vi "Context Owner.vi"() -> ()   [LabVIEW 2019, in "RemoteControl.ZMQ.lvlib" / "ZMQ.ContextManager.lvlib"]
uses:
  ZMQ.ContextManager.lvlib
  Typedefs/Action--enum.ctl
  <vilib>/addons/zeromq/zmq_context.lvclass
panel:
  out "Numeric":i32
  in  "stop":bool
  out "error out":errorcluster
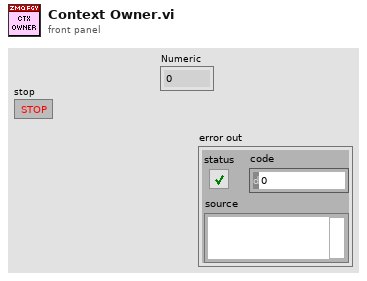
[diagram p1: front panel]
types:
  T1 = typedef "RemoteControl.ZMQ.lvlib/ZMQ.ContextManager.lvlib/Action--enum.ctl" = enum16{"Get Context", "Release Context", "Socket Opened", "Socket Closed", "Force Cleanup", "Set Context", "Retire If Idle"}
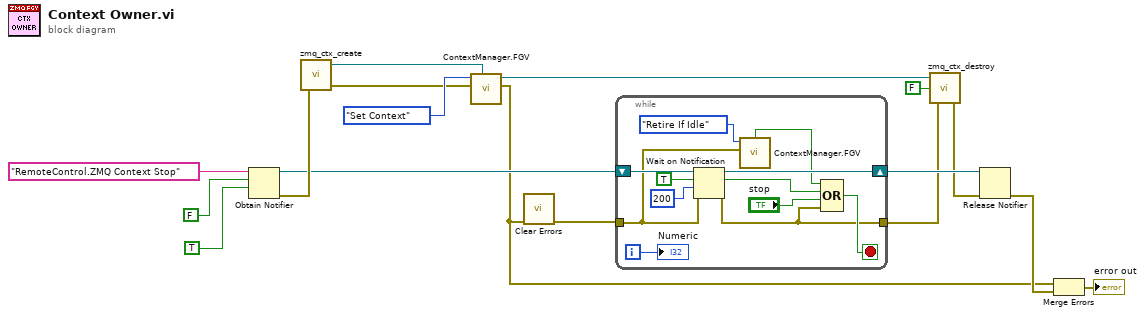
[diagram p0: block diagram]
diagram:
  n1 = Obtain Notifier(name (unnamed)="RemoteControl.ZMQ Context Stop", notification data type=FALSE, create if not found? (T)=TRUE) -> (notifier out=w5:refnum<notifier>, error out=w6:errorcluster)  [unwired: 1 in, 1 out]
  n2 = call <vilib>:"zmq_ctx_create.vi"("error in"=w6) -> ("error out"=w12:errorcluster, "context out"=w14:refnum<class "zmq_context.lvclass">)  [unwired: 3 in]
  n3 = call "ContextManager.FGV.vi"("context in"=w14, "error in"=w12, "action"=Action--enum."Set Context") -> ("error out"=w2:errorcluster, "context out"=w1:refnum<class "zmq_context.lvclass">)  [unwired: 6 in, 1 out]
  n4 = call <vilib>:"Clear Errors.vi"("error in (no error)"=w2) -> ("error out"=w7:errorcluster)  [unwired: 5 in, 1 out]
  n5 = while {
    shift-right: [w28] -> w10
    shift-left: w5 -> [w26]
    tunnel: w7 -> [w20]
    tunnel: [w19] -> w4
    i -> [w21]
    stop <- w24 stop-if-true
    n6 = Wait on Notification(notifier=w26, ignore previous (F)=TRUE, timeout in ms (-1)=200, error in (no error)=w20) -> (notifier out=w28:refnum<notifier>, notification=w25:bool, error out=w19:errorcluster)  [unwired: 1 out]
    n7 = call "ContextManager.FGV.vi"("error in"=w20, "action"=Action--enum."Retire If Idle") -> ("retired?"=w23:bool)  [unwired: 7 in, 2 out]
    n8 = Compound Arithmetic op=OR(w23, w25, "stop", w19) -> (w24:bool)
    "Numeric" <- w21
  }
  n9 = call <vilib>:"zmq_ctx_destroy.vi"("error in"=w4, "reap? (F)"=FALSE, "context in"=w1) -> ("error out"=w3:errorcluster)  [unwired: 2 in]
  n10 = Release Notifier(notifier=w10, error in (no error)=w3) -> (error out=w9:errorcluster)  [unwired: 1 in, 2 out]
  n11 = Merge Errors(w2, w9) -> (→"error out":errorcluster)
